vi "Menu.Sequence.Load.vi"(8 "error in (no error)":errorcluster, 9 "Coords":T1, 10 "MenuRef":refnum<k9>, 11 "State Variables":T2={"Aliases.All"=[], "Aliases.Outputs"=[], "UI.Sequence#ofColumns"=0, "SysDef.Path"=path "", "UI.SequenceRef"=refnum, "UI.StepInformationRef"=refnum, "UI.AbortRef"=refnum, "UI.GraphRef"=refnum, "UI.ViewRef"=refnum, "UI.IterationsRef"=refnum, "UI.IterationInformationRef"=refnum, "INI.Settings"={"Build Location"=path "C:/Simple Sequence Editor/SequenceRepo", "LoggingLocation"=path ""}, "NIVS.Workspace Event"=refnum, "UI.SkipChannel"=refnum, "NIVS.Launched?"=FALSE, "UI.DurationChannel"=refnum}) -> (0 "error out":errorcluster, 3 "State Variables out":T2={"Aliases.All"=[], "Aliases.Outputs"=[], "UI.Sequence#ofColumns"=0, "SysDef.Path"=path "", "UI.SequenceRef"=refnum, "UI.StepInformationRef"=refnum, "UI.AbortRef"=refnum, "UI.GraphRef"=refnum, "UI.ViewRef"=refnum, "UI.IterationsRef"=refnum, "UI.IterationInformationRef"=refnum, "INI.Settings"={"Build Location"=path "C:/Simple Sequence Editor/SequenceRepo", "LoggingLocation"=path ""}, "NIVS.Workspace Event"=refnum, "UI.SkipChannel"=refnum, "NIVS.Launched?"=FALSE, "UI.DurationChannel"=refnum})   [LabVIEW 2015, in "Simple Sequence Tools - Editor.lvlib"]
uses:
  Simple Sequence Tools - Editor.lvlib
  Types/Main.StateVariables.ctl
  Shared/Types/Channel.Properties.ctl
  Shared/Types/INI.Settings.ctl
  <vilib>/Utility/miscctls.llb/LVPoint32TypeDef.ctl
  Shared/SubVIs/Main.Constants.vi
  Shared/Simple Sequence Tools - Shared.lvlib
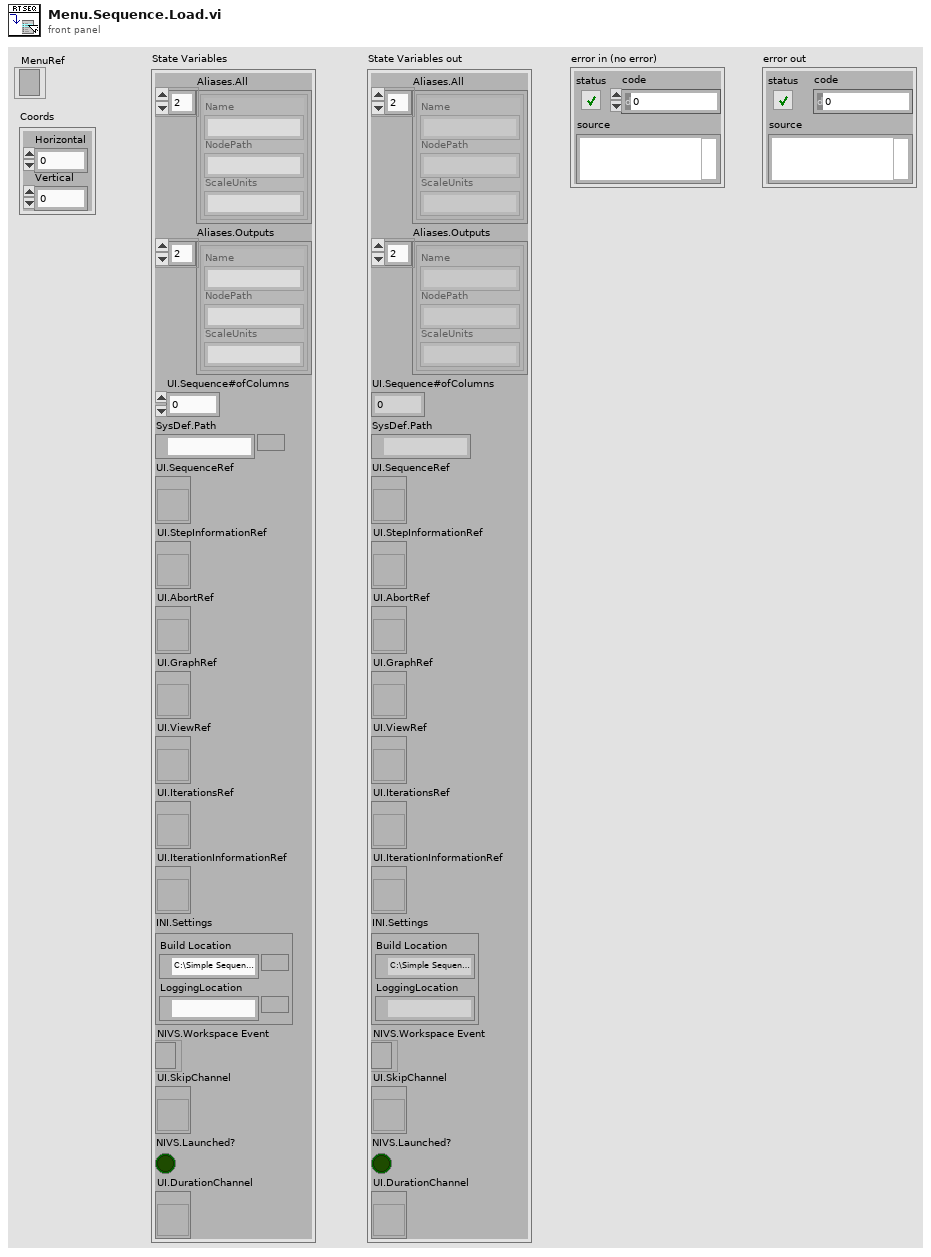
[diagram p1: front panel]
types:
  T1 = typedef "LVPoint32TypeDef.ctl" = cluster{"Horizontal":i32, "Vertical":i32}
  T2 = typedef "Simple Sequence Tools - Editor.lvlib/Main.StateVariables.ctl" = cluster{"Aliases.All":T3[], "Aliases.Outputs":T3[], "UI.Sequence#ofColumns":i32, "SysDef.Path":path, "UI.SequenceRef":refnum<vi>, "UI.StepInformationRef":refnum<vi>, "UI.AbortRef":refnum<vi>, "UI.GraphRef":refnum<vi>, "UI.ViewRef":refnum<vi>, "UI.IterationsRef":refnum<vi>, "UI.IterationInformationRef":refnum<vi>, "INI.Settings":T4, "NIVS.Workspace Event":refnum<event-registration>, "UI.SkipChannel":refnum<vi>, "NIVS.Launched?":bool, "UI.DurationChannel":refnum<vi>}
  T3 = typedef "Simple Sequence Tools - Shared.lvlib/Channel.Properties.ctl" = cluster{"Name":string, "NodePath":string, "ScaleUnits":string}
  T4 = typedef "Simple Sequence Tools - Shared.lvlib/INI.Settings.ctl" = cluster{"Build Location":path, "LoggingLocation":path}
  T5 = typedef "LVRowAndColumnTypeDef.ctl" = cluster{"Row":i32, "Column":i32}
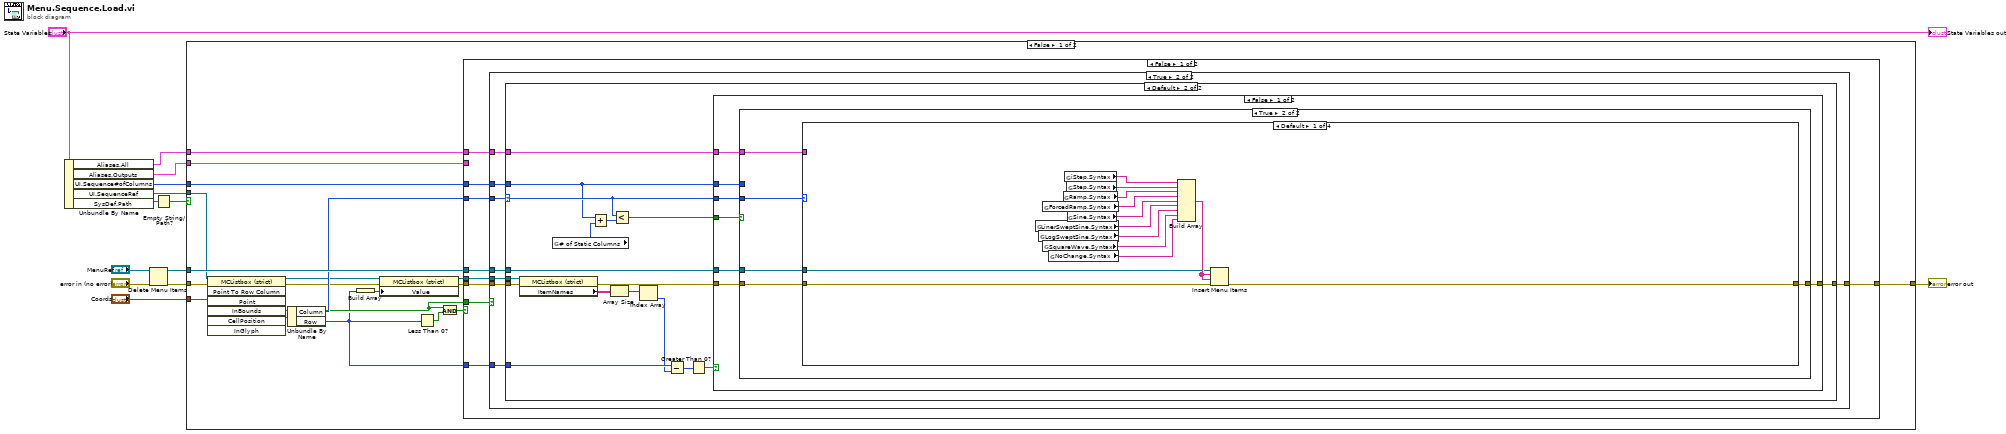
[diagram p0: block diagram]
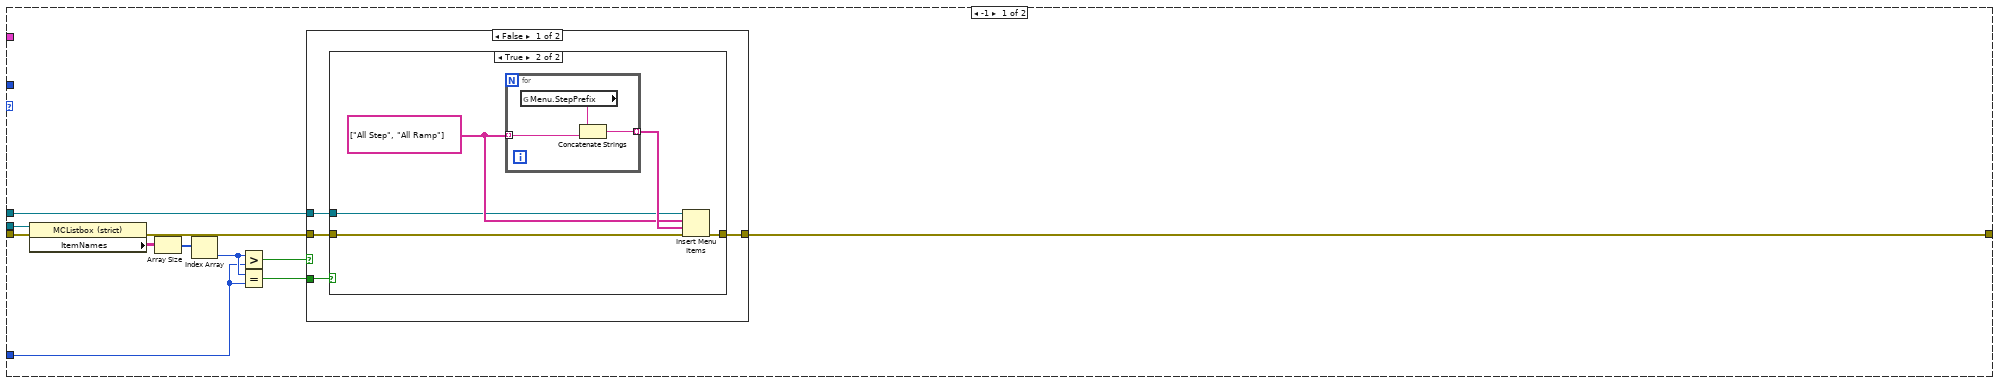
[diagram p3: hidden frame]
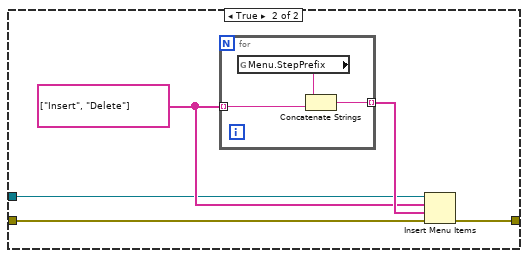
[diagram p5: hidden frame]
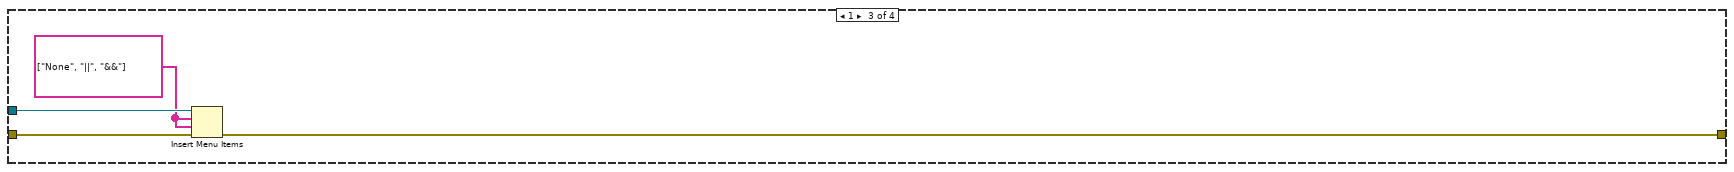
[diagram p8: hidden frame]
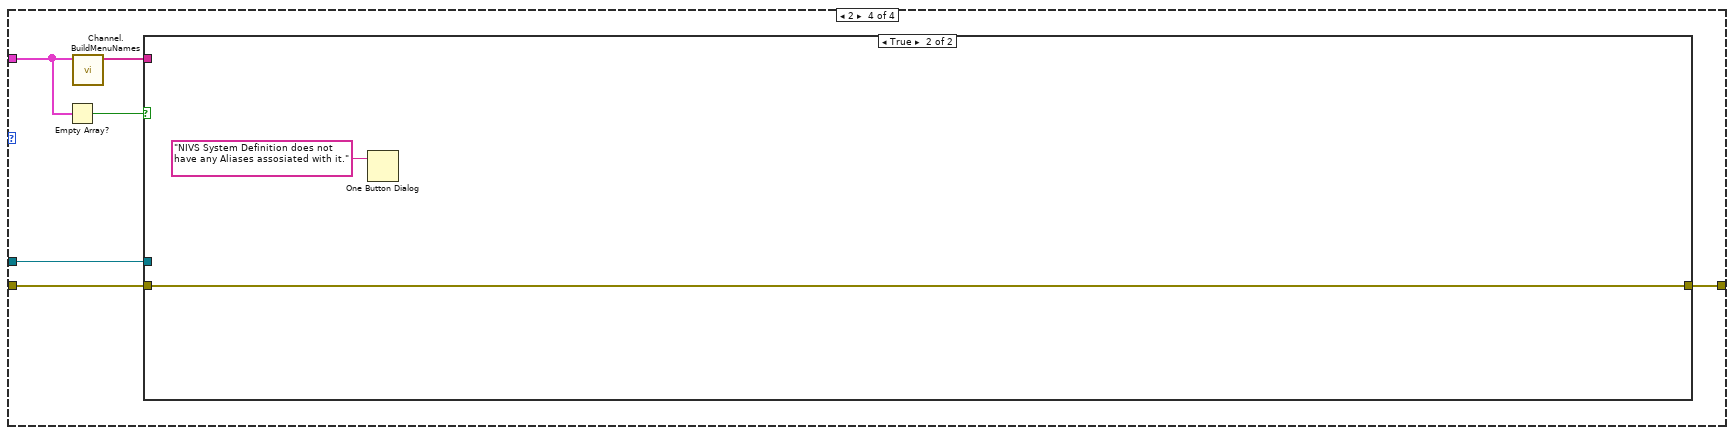
[diagram p9: hidden frame]
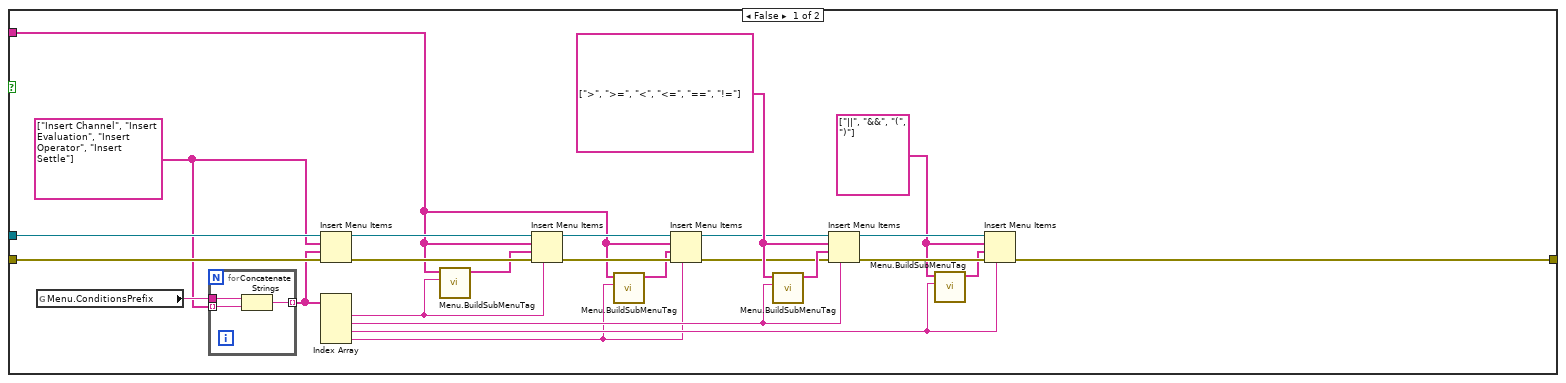
[diagram p10: hidden frame]
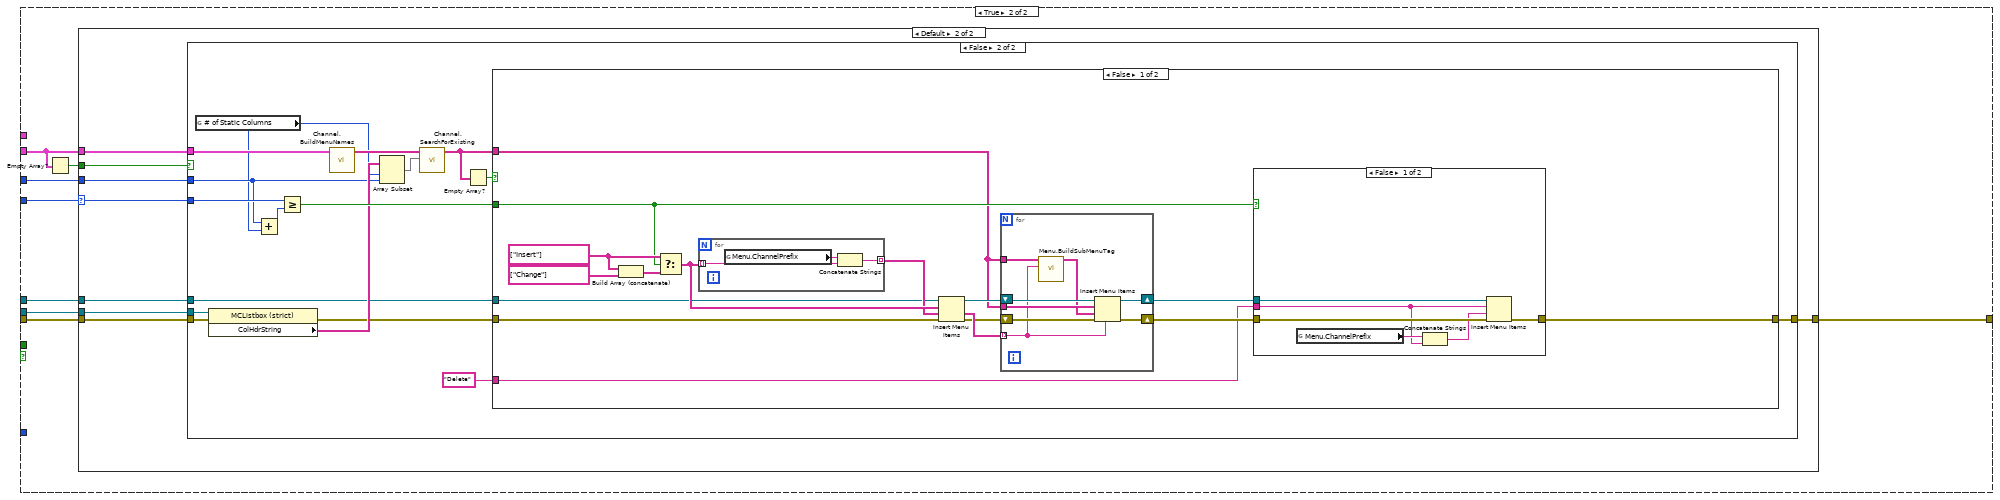
[diagram p12: hidden frame]
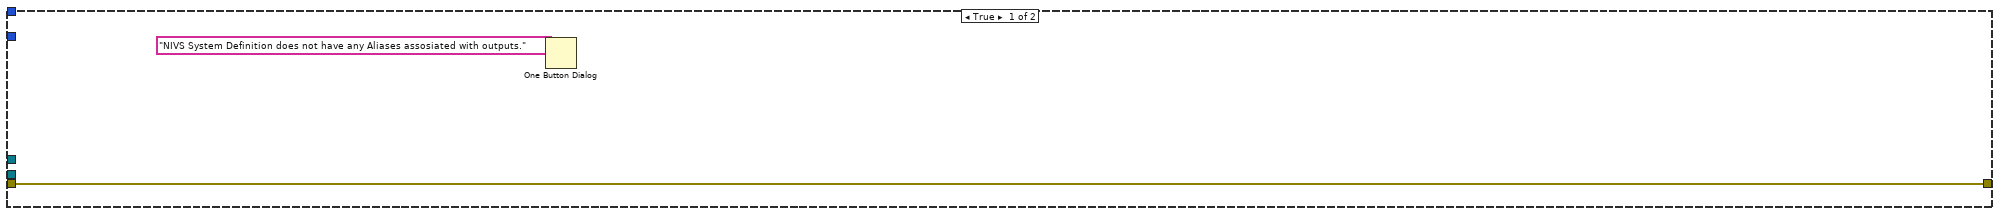
[diagram p14: hidden frame]
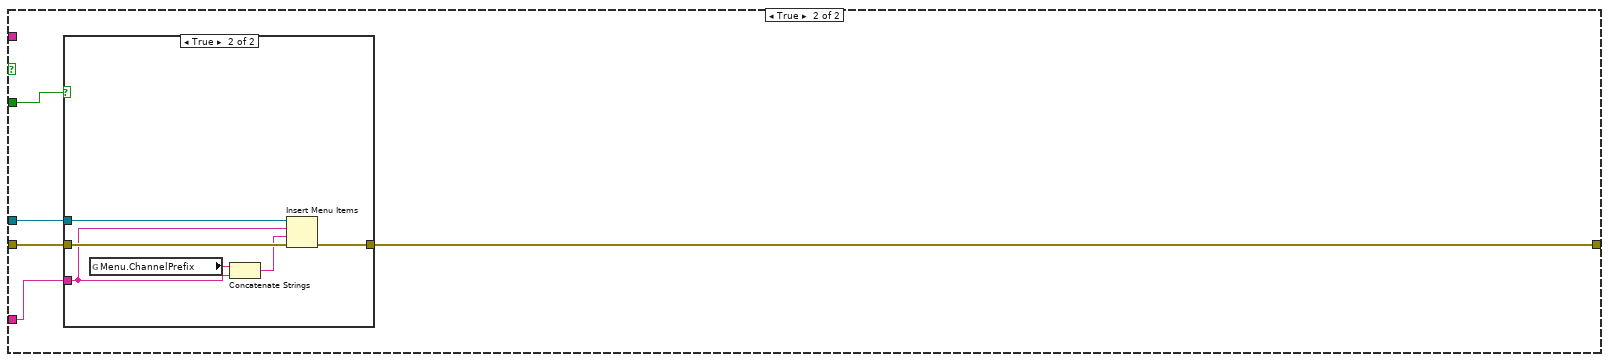
[diagram p16: hidden frame]
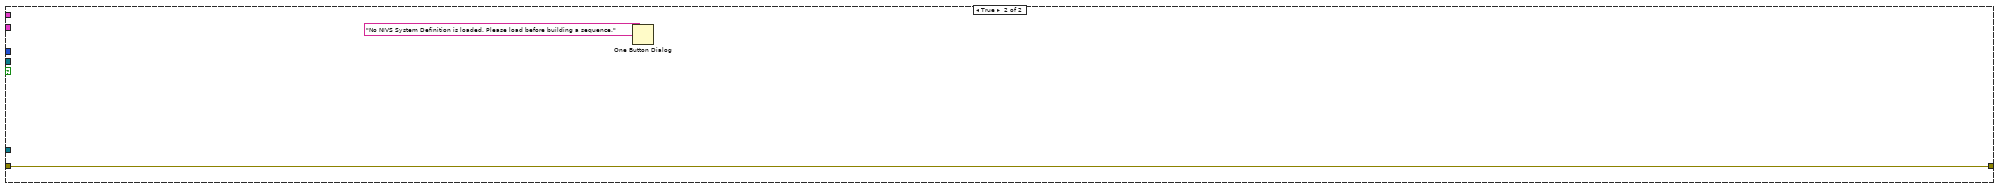
[diagram p18: hidden frame]
diagram:
  n1 = Unbundle By Name("State Variables") -> ("Aliases.All"=w1:T3[], "Aliases.Outputs"=w9:T3[], "UI.Sequence#ofColumns"=w12:i32, "UI.SequenceRef"=w10:refnum<vi>, "SysDef.Path"=w7:path)
  n2 = Delete Menu Items(6:"error in (no error)", 9:"MenuRef") -> (0:w4:errorcluster, 3:w2:refnum<k9>)  [unwired: 2 in]
  n3 = Empty String/Path?(string/path=w7) -> (empty?=w6:bool)
  n4 = case shown="False" w6 {
    tunnel: [w32 w250] -> w13
    tunnel: w2 -> [w31 _]
    tunnel: w12 -> [w30 _]
    tunnel: "Coords" -> [w25 _]
    tunnel: w10 -> [w24 _]
    tunnel: w4 -> [w23 w250]
    tunnel: w9 -> [w22 _]
    tunnel: w1 -> [w20 _]
    frame False {
      n5 = invoke class="MCListbox (strict)" method="Point To Row Column"(reference=w24, error in=w23, "Point"=w25) -> (reference out=w18:refnum<vi>, error out=w19:errorcluster, "InBounds"=w21:bool, "CellPosition"=w26:T5)  [unwired: 4 in, 3 out]
      n6 = Unbundle By Name(w26) -> ("Column"=w29:i32, "Row"=w15:i32)
      n7 = Build Array(w15) -> (w14:i32[])
      n8 = property class="MCListbox (strict)"(reference=w18, error in=w19, "Value"=w14) -> (reference out=w16:refnum<vi>, error out=w17:errorcluster)
      n9 = Less Than 0?(x=w15) -> (x < 0?=w27:bool)
      n10 = And(x=w21, y=w27) -> (x .and. y?=w28:bool)
      n11 = case shown="False" w28 {
        tunnel: w29 -> [w36 w168]
        tunnel: w30 -> [w37 w169]
        tunnel: w31 -> [w35 w172]
        tunnel: w17 -> [w40 w173]
        tunnel: [w34 w174] -> w32
        tunnel: w16 -> [w39 w175]
        tunnel: w22 -> [_ w171]
        tunnel: w21 -> [w41 _]
        tunnel: w15 -> [w38 _]
        tunnel: w20 -> [w33 _]
        frame False {
          n12 = case shown="True" w41 {
            tunnel: w40 -> [w42 w49]
            tunnel: w39 -> [_ w50]
            tunnel: w38 -> [_ w48]
            tunnel: w37 -> [_ w47]
            tunnel: w36 -> [_ w46]
            tunnel: w35 -> [_ w45]
            tunnel: [w42 w44] -> w34
            tunnel: w33 -> [_ w43]
            frame False {
            }
            frame True {
              n13 = case shown="Default" w46 {
                selector: w46 -> [_ w90]
                tunnel: w50 -> [w57 w99]
                tunnel: w49 -> [w59 w98]
                tunnel: w48 -> [w52 w95]
                tunnel: w47 -> [_ w84]
                tunnel: w45 -> [w60 w91]
                tunnel: [w61 w88] -> w44
                tunnel: w43 -> [_ w86]
                frame -1 {
                  n14 = property class="MCListbox (strict)"(reference=w57, error in=w59) -> (error out=w58:errorcluster, "ItemNames"=w55:string[][])  [unwired: 1 out]
                  n15 = Array Size(array=w55) -> (size(s)=w56:i32[])
                  n16 = Index Array(array=w56) -> (element=w53:i32)  [unwired: 1 in]
                  n17 = Greater?(x=w53, y=w52) -> (0:w54:bool)
                  n18 = Equal?(x=w53, y=w52) -> (x = y?=w51:bool)
                  n19 = case shown="False" w54 {
                    tunnel: [w64 w79] -> w61
                    tunnel: w60 -> [w63 w76]
                    tunnel: w58 -> [w65 w75]
                    tunnel: w51 -> [w62 _]
                    frame False {
                      n20 = case shown="True" w62 {
                        tunnel: w65 -> [w66 w69]
                        tunnel: [w66 w68] -> w64
                        tunnel: w63 -> [_ w67]
                        frame False {
                        }
                        frame True {
                          w70 = string[] ["All Step", "All Ramp"] ("item names")
                          n21 = for {
                            tunnel: [w73] -> w71 mode=indexing
                            tunnel: w70 -> [w74] mode=indexing
                            n22 = global read "Main.Constants.vi" "Menu.StepPrefix"() -> (w72:string)
                            n23 = Concatenate Strings(w72, w74) -> (w73:string)
                          }
                          n24 = Insert Menu Items(6:w69, 7:w71, 8:w70, 9:w67) -> (0:w68:errorcluster)  [unwired: 2 in, 2 out]
                        }
                      }
                    }
                    frame True {
                      w77 = string[] ["Insert", "Delete"] ("item names")
                      n25 = for {
                        tunnel: [w81] -> w78 mode=indexing
                        tunnel: w77 -> [w82] mode=indexing
                        n26 = global read "Main.Constants.vi" "Menu.StepPrefix"() -> (w80:string)
                        n27 = Concatenate Strings(w80, w82) -> (w81:string)
                      }
                      n28 = Insert Menu Items(6:w75, 7:w78, 8:w77, 9:w76) -> (0:w79:errorcluster)  [unwired: 2 in, 2 out]
                    }
                  }
                }
                frame Default {
                  n29 = property class="MCListbox (strict)"(reference=w99, error in=w98) -> (error out=w93:errorcluster, "ItemNames"=w97:string[][])  [unwired: 1 out]
                  n30 = global read "Main.Constants.vi" "# of Static Columns"() -> (w85:u32)
                  n31 = Add(x=w84, y=w85) -> (x+y=w83:u32)
                  n32 = Array Size(array=w97) -> (size(s)=w96:i32[])
                  n33 = Less?(x=w90, y=w83) -> (x < y?=w89:bool)
                  n34 = Index Array(array=w96) -> (element=w94:i32)  [unwired: 1 in]
                  n35 = Subtract(x=w95, y=w94) -> (x-y=w87:i32)
                  n36 = Greater Than 0?(x=w87) -> (x > 0?=w92:bool)
                  n37 = case shown="False" w92 {
                    tunnel: w93 -> [w106 w167]
                    tunnel: w84 -> [w103 _]
                    tunnel: w90 -> [w102 _]
                    tunnel: w91 -> [w105 _]
                    tunnel: w89 -> [w104 _]
                    tunnel: [w101 w167] -> w88
                    tunnel: w86 -> [w100 _]
                    frame False {
                      n38 = case shown="True" w104 {
                        tunnel: w106 -> [w107 w111]
                        tunnel: w105 -> [_ w112]
                        tunnel: w103 -> [_ _]
                        tunnel: w102 -> [_ w108]
                        tunnel: [w107 w110] -> w101
                        tunnel: w100 -> [_ w109]
                        frame False {
                        }
                        frame True {
                          n39 = case shown="Default" w108 {
                            tunnel: w112 -> [w114 _ w130 w136]
                            tunnel: w111 -> [w116 w126 w129 w135]
                            tunnel: [w115 w126 w127 w134] -> w110
                            tunnel: w109 -> [_ _ _ w133]
                            frame Default {
                              n40 = global read "Main.Constants.vi" "LinerSweptSine.Syntax"() -> (w120:string)
                              n41 = global read "Main.Constants.vi" "LogSweptSine.Syntax"() -> (w117:string)
                              n42 = global read "Main.Constants.vi" "ForcedRamp.Syntax"() -> (w118:string)
                              n43 = global read "Main.Constants.vi" "SquareWave.Syntax"() -> (w113:string)
                              n44 = global read "Main.Constants.vi" "NoChange.Syntax"() -> (w123:string)
                              n45 = global read "Main.Constants.vi" "Ramp.Syntax"() -> (w119:string)
                              n46 = global read "Main.Constants.vi" "iStep.Syntax"() -> (w122:string)
                              n47 = global read "Main.Constants.vi" "Step.Syntax"() -> (w125:string)
                              n48 = global read "Main.Constants.vi" "Sine.Syntax"() -> (w121:string)
                              n49 = Build Array(w122, w125, w119, w118, w121, w120, w117, w113, w123) -> (w124:string[])
                              n50 = Insert Menu Items(6:w116, 7:w124, 8:w124, 9:w114) -> (0:w115:errorcluster)  [unwired: 2 in, 2 out]
                            }
                            frame 0 {
                            }
                            frame 1 {
                              w128 = string[] ["None", "||", "&&"] ("item names")
                              n51 = Insert Menu Items(6:w129, 7:w128, 8:w128, 9:w130) -> (0:w127:errorcluster)  [unwired: 2 in, 2 out]
                            }
                            frame 2 {
                              n52 = Empty Array?(array=w133) -> (empty?=w132:bool)
                              n53 = call "Channel.BuildMenuNames.vi"("Aliases"=w133) -> ("Aliases Array"=w131:string[])  [unwired: 10 in]
                              n54 = case shown="True" w132 {
                                tunnel: w136 -> [w161 _]
                                tunnel: w135 -> [w160 w165]
                                tunnel: [w145 w165] -> w134
                                tunnel: w131 -> [w138 _]
                                frame False {
                                w147 = string[] [">", ">=", "<", "<=", "==", "!="] ("item names")
                                w146 = string[] ["||", "&&", "(", ")"] ("item names")
                                w158 = string[] ["Insert Channel", "Insert Evaluation", "Insert Operator", "Insert Settle"] ("item names")
                                n55 = global read "Main.Constants.vi" "Menu.ConditionsPrefix"() -> (w159:string)
                                n56 = for {
                                tunnel: w158 -> [w164] mode=indexing
                                tunnel: w159 -> [w163]
                                tunnel: [w162] -> w154 mode=indexing
                                n57 = Concatenate Strings(w163, w164) -> (w162:string)
                                }
                                n58 = Insert Menu Items(6:w160, 7:w154, 8:w158, 9:w161) -> (0:w157:errorcluster, 3:w156:refnum<k9>)  [unwired: 2 in, 1 out]
                                n59 = Index Array(array=w154) -> (element #1=w155:string, element #2=w151:string, element #3=w149:string, element #4=w137:string)  [unwired: 4 in]
                                n60 = call "Menu.BuildSubMenuTag.vi"("Menu"=w155, "Aliases Array"=w138) -> ("Tag Array"=w140:string[])  [unwired: 9 in]
                                n61 = Insert Menu Items(5:w155, 6:w157, 7:w140, 8:w138, 9:w156) -> (0:w144:errorcluster, 3:w142:refnum<k9>)  [unwired: 1 in, 1 out]
                                n62 = call "Menu.BuildSubMenuTag.vi"("Menu"=w137, "Aliases Array"=w138) -> ("Tag Array"=w139:string[])  [unwired: 9 in]
                                n63 = Insert Menu Items(5:w137, 6:w144, 7:w139, 8:w138, 9:w142) -> (0:w143:errorcluster, 3:w141:refnum<k9>)  [unwired: 1 in, 1 out]
                                n64 = call "Menu.BuildSubMenuTag.vi"("Menu"=w151, "Aliases Array"=w147) -> ("Tag Array"=w150:string[])  [unwired: 9 in]
                                n65 = Insert Menu Items(5:w151, 6:w143, 7:w150, 8:w147, 9:w141) -> (0:w153:errorcluster, 3:w152:refnum<k9>)  [unwired: 1 in, 1 out]
                                n66 = call "Menu.BuildSubMenuTag.vi"("Menu"=w149, "Aliases Array"=w146) -> ("Tag Array"=w148:string[])  [unwired: 9 in]
                                n67 = Insert Menu Items(5:w149, 6:w153, 7:w148, 8:w146, 9:w152) -> (0:w145:errorcluster)  [unwired: 1 in, 2 out]
                                }
                                frame True {
                                n68 = One Button Dialog(message="NIVS System Definition does not have any Aliases assosiated with it.") -> ()  [unwired: 1 in, 1 out]
                                }
                              }
                            }
                          }
                        }
                      }
                    }
                    frame True {
                    }
                  }
                }
              }
            }
          }
        }
        frame True {
          n69 = Empty Array?(array=w171) -> (empty?=w170:bool)
          n70 = case shown="Default" w168 {
            selector: w168 -> [_ w177]
            tunnel: w175 -> [_ w184]
            tunnel: [w176 w183] -> w174
            tunnel: w173 -> [w176 w182]
            tunnel: w172 -> [_ w181]
            tunnel: w171 -> [_ w180]
            tunnel: w170 -> [_ w179]
            tunnel: w169 -> [_ w178]
            frame -1..2 {
            }
            frame Default {
              n71 = case shown="False" w179 {
                tunnel: w177 -> [_ w190]
                tunnel: w184 -> [_ w202]
                tunnel: w178 -> [_ w189]
                tunnel: [w186 w200] -> w183
                tunnel: w180 -> [_ w199]
                tunnel: w182 -> [w186 w195]
                tunnel: w181 -> [_ w196]
                frame True {
                  n72 = One Button Dialog(message="NIVS System Definition does not have any Aliases assosiated with outputs.") -> ()  [unwired: 1 in, 1 out]
                }
                frame False {
                  n73 = global read "Main.Constants.vi" "# of Static Columns"() -> (w188:u32)
                  n74 = property class="MCListbox (strict)"(reference=w202, error in=w195) -> (error out=w194:errorcluster, "ColHdrString"=w201:string[])  [unwired: 1 out]
                  n75 = Add(x=w189, y=w188) -> (x+y=w187:u32)
                  n76 = Greater Or Equal?(x=w190, y=w187) -> (x >= y?=w203:bool)
                  n77 = call "Channel.BuildMenuNames.vi"("Aliases"=w199) -> ("Aliases Array"=w197:string[])  [unwired: 10 in]
                  n78 = Array Subset(array=w201, index=w188, length=w189) -> (w198:string[])
                  n79 = call "Channel.SearchForExisting.vi"("Existing Channels"=w198, "All Channels"=w197) -> ("Array out"=w193:string[])  [unwired: 9 in]
                  n80 = Empty Array?(array=w193) -> (empty?=w192:bool)
                  n81 = case shown="False" w192 {
                    tunnel: w203 -> [w205 w238]
                    tunnel: [w208 w241] -> w200
                    tunnel: w196 -> [w212 w240]
                    tunnel: w193 -> [w204 _]
                    tunnel: w194 -> [w210 w242]
                    tunnel: "Delete" ("string") -> [w206 w239]
                    frame False {
                      w217 = string[] ["Insert"]
                      n82 = Build Array (concatenate)(w217, string[] ["Change"]) -> (w218:string[])
                      n83 = Select(t=w217, s=w205, f=w218) -> (s? t:f=w216:string[])
                      n84 = for {
                        tunnel: w216 -> [w237] mode=indexing
                        tunnel: [w236] -> w215 mode=indexing
                        n85 = global read "Main.Constants.vi" "Menu.ChannelPrefix"() -> (w235:string)
                        n86 = Concatenate Strings(w235, w237) -> (w236:string)
                      }
                      n87 = Insert Menu Items(6:w210, 7:w215, 8:w216, 9:w212) -> (0:w211:errorcluster, 1:w213:string[], 3:w214:refnum<k9>)  [unwired: 2 in]
                      n88 = for {
                        tunnel: w213 -> [w229] mode=indexing
                        shift-right: [w233] -> w209
                        shift-left: w211 -> [w234]
                        tunnel: w204 -> [w231]
                        shift-right: [w230] -> w207
                        shift-left: w214 -> [w232]
                        tunnel: w204 -> [w228]
                        n89 = call "Menu.BuildSubMenuTag.vi"("Menu"=w229, "Aliases Array"=w228) -> ("Tag Array"=w227:string[])  [unwired: 9 in]
                        n90 = Insert Menu Items(5:w229, 6:w234, 7:w227, 8:w231, 9:w232) -> (0:w233:errorcluster, 3:w230:refnum<k9>)  [unwired: 1 in, 1 out]
                      }
                      n91 = case shown="False" w205 {
                        tunnel: w209 -> [w225 w226]
                        tunnel: [w224 w226] -> w208
                        tunnel: w207 -> [w223 _]
                        tunnel: w206 -> [w220 _]
                        frame False {
                          n92 = global read "Main.Constants.vi" "Menu.ChannelPrefix"() -> (w222:string)
                          n93 = Concatenate Strings(w222, w220) -> (w221:string)
                          n94 = Insert Menu Items(6:w225, 7:w221, 8:w220, 9:w223) -> (0:w224:errorcluster)  [unwired: 2 in, 2 out]
                        }
                        frame True {
                        }
                      }
                    }
                    frame True {
                      n95 = case shown="True" w238 {
                        tunnel: w242 -> [w243 w249]
                        tunnel: [w243 w248] -> w241
                        tunnel: w240 -> [_ w247]
                        tunnel: w239 -> [_ w245]
                        frame False {
                        }
                        frame True {
                          n96 = global read "Main.Constants.vi" "Menu.ChannelPrefix"() -> (w246:string)
                          n97 = Concatenate Strings(w246, w245) -> (w244:string)
                          n98 = Insert Menu Items(6:w249, 7:w244, 8:w245, 9:w247) -> (0:w248:errorcluster)  [unwired: 2 in, 2 out]
                        }
                      }
                    }
                  }
                }
              }
            }
          }
        }
      }
    }
    frame True {
      n99 = One Button Dialog(message="No NIVS System Definition is loaded. Please load before building a sequence.") -> ()  [unwired: 1 in, 1 out]
    }
  }
  "error out" <- w13
  "State Variables out" <- "State Variables"
